vi "DAC Run.vi"(8 "error in":errorcluster, 11 "DAC HeatFlow Load dU in":refnum<class "DAC HeatFlow Load dU.lvclass">) -> (0 "error out":errorcluster, 3 "DAC HeatFlow Load dU out":refnum<class "DAC HeatFlow Load dU.lvclass">)   [LabVIEW 2019, in "DAC.lvlib" / "DAC HeatFlow Load dU.lvclass"]
uses:
  DAC HeatFlow Load dU.lvclass
  C:/Users/krio/Documents/LV_Projects/test-stand/App/DAC/DAC.lvclass
  DAC.lvclass/DAC.ctl
  Results/Results Method.ctl
  Results/Heat Flow Results/Heat Flow Results.lvclass
  DAC HeatFlow Load dU.lvclass/DAC HeatFlow Load dU.ctl
  Results/Heat Flow Results/Heat Flow Results.lvclass/Heat Flow Results.ctl
  <vilib>/DAQmx/read.llb/DAQmx Read (Analog DBL 1Chan 1Samp).vi
  <vilib>/DAQmx/miscellaneous.llb/DAQmx Fill In Error Info.vi
  DAC.lvclass
  Results/Results.lvlib
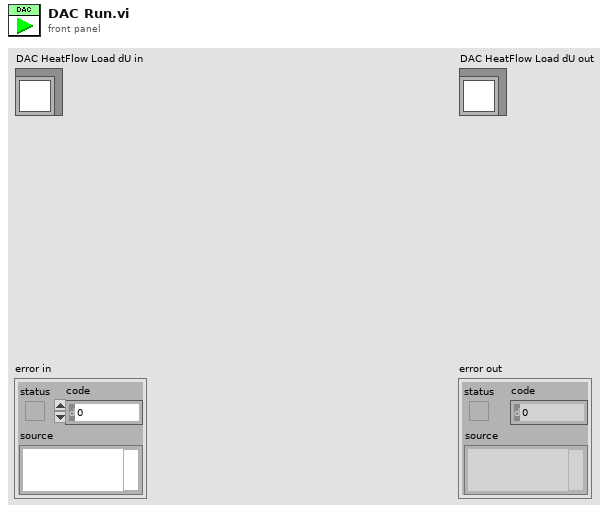
[diagram p1: front panel]
types:
  T1 = typedef "Results.lvlib/Results Method.ctl" = enum16{"Get", "Set"}
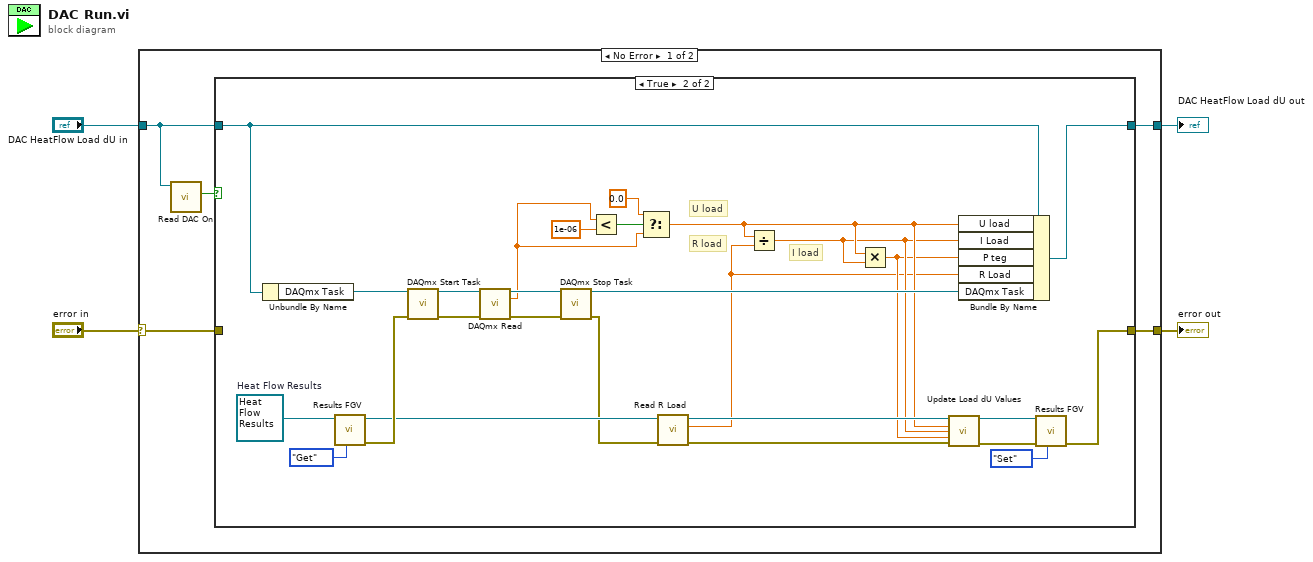
[diagram p0: block diagram]
diagram:
  n1 = case shown="No Error" "error in" {
    selector: "error in" -> [w7 w40]
    tunnel: [w6 w40] -> w2
    tunnel: [w8 w39] -> w1
    tunnel: "DAC HeatFlow Load dU in" -> [w5 w39]
    frame No Error {
      n2 = call "Read DAC On.vi"("DAC in"=w5) -> ("DAC On"=w9:bool)  [unwired: 8 in, 2 out]
      n3 = case shown="True" w9 {
        tunnel: w5 -> [w11 w37]
        tunnel: [w11 w38] -> w8
        tunnel: w7 -> [w10 _]
        tunnel: [w10 w25] -> w6
        frame False {
        }
        frame True {
          w30 = refnum<class "Heat Flow Results.lvclass"> refnum  # Heat Flow Results
          # "I load"
          # "R load"
          # "U load"
          n4 = Unbundle By Name(w37) -> ("DAQmx Task"=w27:refnum<k21>)
          n5 = call-dynamic "Results FGV.vi"("Method"=Results_Method."Get", "Results in"=w30) -> ("error out"=w29:errorcluster, "Results out"=w22:refnum<class "Heat Flow Results.lvclass">)  [unwired: 8 in]
          n6 = call <vilib>:"DAQmx Start Task.vi"("task/channels in"=w27, "error in"=w29) -> ("task out"=w36:refnum<k21>, "error out"=w34:errorcluster)  [unwired: 12 in]
          n7 = call-poly <vilib>:"DAQmx Read.vi"("task/channels in"=w36, "error in"=w34) -> ("task out"=w35:refnum<k21>, "data"=w28:dbl, "error out"=w33:errorcluster)  [unwired: 11 in]
          n8 = call <vilib>:"DAQmx Stop Task.vi"("task/channels in"=w35, "error in"=w33) -> ("task out"=w26:refnum<k21>, "error out"=w16:errorcluster)  [unwired: 12 in]
          n9 = Less?(x=w28, y=1e-06) -> (x < y?=w13:bool)
          n10 = Select(t=0.0, s=w13, f=w28) -> (s? t:f=w20:dbl)
          n11 = call "Read R Load.vi"("error in (no error)"=w16, "Heat Flow Results in"=w22) -> ("error out"=w15:errorcluster, "R Load"=w17:dbl, "Heat Flow Results out"=w21:refnum<class "Heat Flow Results.lvclass">)  [unwired: 7 in]
          n12 = Divide(x=w20, y=w17) -> (x/y=w19:dbl)
          n13 = Multiply(x=w20, y=w19) -> (x*y=w18:dbl)
          n14 = call "Update Load dU Values.vi"("Heat Flow Results in"=w21, "R load U"=w20, "I Load"=w19, "P_teg"=w18, "error in"=w15) -> ("Heat Flow Results out"=w23:refnum<class "Heat Flow Results.lvclass">, "error out"=w24:errorcluster)  [unwired: 9 in]
          n15 = Bundle By Name(cluster=w37, "U load"=w20, "I Load"=w19, "P teg"=w18, "R Load"=w17, "DAQmx Task"=w26) -> (w38:refnum<class "DAC HeatFlow Load dU.lvclass">)
          n16 = call-dynamic "Results FGV.vi"("Method"=Results_Method."Set", "error in"=w24, "Results in"=w23) -> ("error out"=w25:errorcluster)  [unwired: 7 in, 1 out]
        }
      }
    }
    frame Error {
    }
  }
  "error out" <- w2
  "DAC HeatFlow Load dU out" <- w1
